vi "Save Buffer Probe.vi"(0 "vi path":string, 5 "out path":string) -> (4 "status":bool, 15 "error out":errorcluster)   [LabVIEW 2026]
doc: "Open a VI by path, ask LabVIEW for the bytes it would write on save (Save.To Buffer) without saving anything, and write those bytes to out path. Comparing that buffer's linker tables with the file on disk shows whether loading changed what LabVIEW wants to persist."
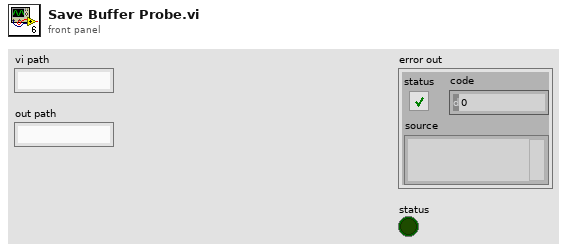
[diagram p1: front panel]
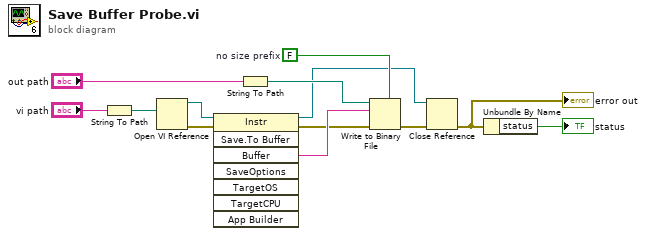
[diagram p0: block diagram]
diagram:
  w5 = FALSE  # no size prefix
  n1 = String To Path(string="vi path") -> (path=w11:path)
  n2 = Open VI Reference(vi path=w11) -> (vi reference=w10:refnum<vi>, error out=w9:errorcluster)  [unwired: 5 in]
  n3 = invoke class="Instr" method="Save.To Buffer"(reference=w10, error in=w9) -> (reference out=w4:refnum<vi>, error out=w6:errorcluster, "Buffer"=w7:string)  [unwired: 6 in, 5 out]
  n4 = String To Path(string="out path") -> (path=w8:path)
  n5 = Write to Binary File(file (use dialog)=w8, data=w7, error in=w6, 5:w5) -> (error out=w3:errorcluster)  [unwired: 2 in, 2 out]
  n6 = Close Reference(reference=w4, error in (no error)=w3) -> (error out=w2:errorcluster)
  "error out" <- w2
  n7 = Unbundle By Name(w2) -> ("status"=→"status":bool)
